vi "Modbus Slave Testbench.vi"() -> ()   [LabVIEW 2021]
uses:
  <vilib>/numeric/Random Number (Range) DBL.vi
  <vilib>/NI/Modbus Library/API/Wrapper/Create TCP Slave.vi
  <vilib>/NI/Modbus Library/API/Slave/Modbus Slave.lvclass
  <vilib>/NI/Modbus Library/API/Wrapper/API Main.lvlib
panel:
  in  "Heatsink Temp (P00022)":u16
  in  "Drive State (P00006)":u16
  in  "DC Link Voltage (P00004)":u16
  in  "Alarm (P00030)":u16
  in  "Fault (P00035)":u16
  out "Fault Reset":u16
  out "Active Mode P00202":enum16{"Nothing", "Torque", "Speed"}(ring)
  out "Command_AO_Reg Setpoint":i16
  out "P00101 Decel":u16
  out "P00100 Accel":u16
  out "Drive Enabled (P00099)":bool
  in  "stop":bool
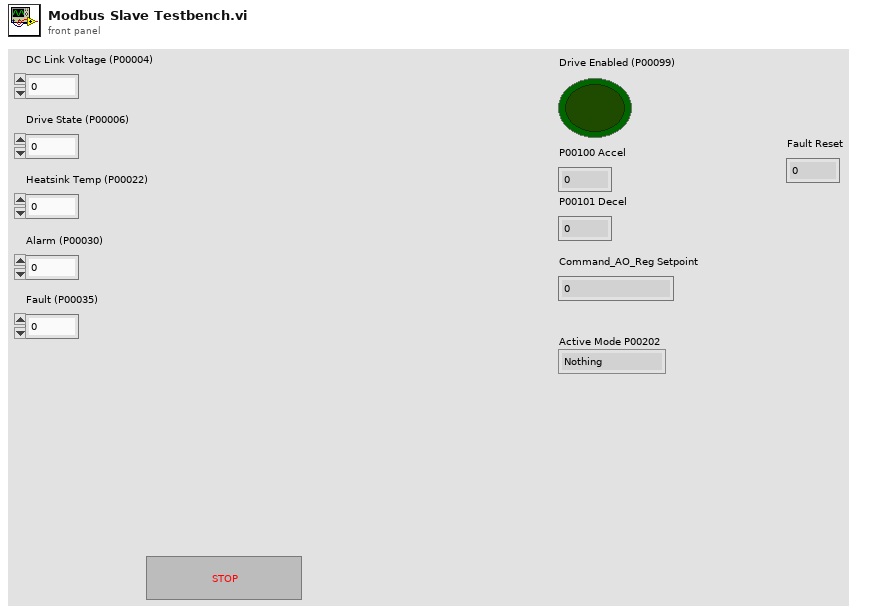
[diagram p1: front panel]
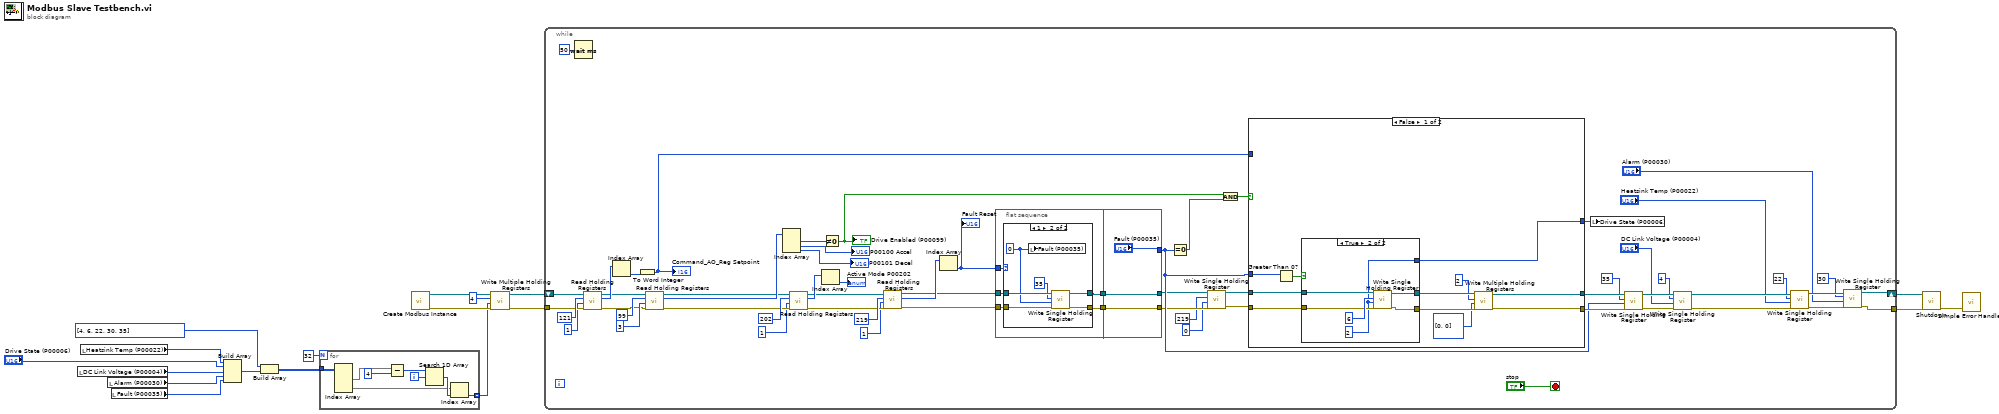
[diagram p0: block diagram]
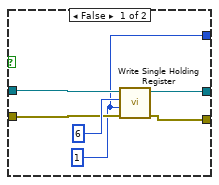
[diagram p3: hidden frame]
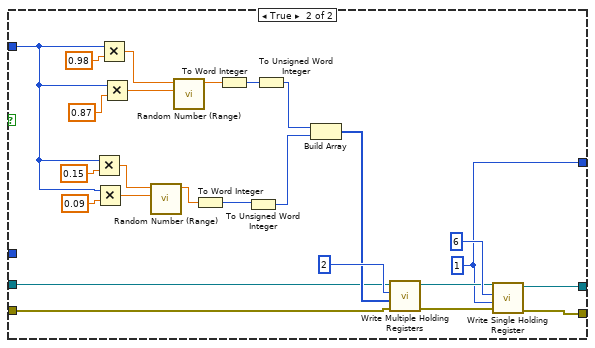
[diagram p4: hidden frame]
diagram:
  n1 = local read "DC Link Voltage (P00004)"() -> (w7:u16)
  n2 = local read "Heatsink Temp (P00022)"() -> (w8:u16)
  n3 = local read "Alarm (P00030)"() -> (w6:u16)
  n4 = local read "Fault (P00035)"() -> (w5:u16)
  n5 = Build Array(w8, "Drive State (P00006)", w7, w6, w5) -> (w3:u16[])
  n6 = Build Array(u16[] [4, 6, 22, 30, 35] ("Simulation Fault"), w3) -> (w2:u16[][])
  n7 = for {
    N: 32 -> [_]
    tunnel: w2 -> [w26]
    tunnel: [w21] -> w12 mode=indexing
    i -> [w24]
    n8 = Index Array(array=w26) -> (element #1=w25:u16[], element #2=w22:u16[])  [unwired: 4 in]
    n9 = Subtract(x=w25, y=4 ("starting address")) -> (x-y=w20:i32[])
    n10 = Search 1D Array(1D array=w20, element=w24) -> (index of element=w23:i32)  [unwired: 1 in]
    n11 = Index Array(array=w22, index=w23) -> (element=w21:u16)
  }
  n12 = call-poly <vilib>:"Create Modbus Instance.vi"() -> ("error out"=w17:errorcluster, "TCP slave instance"=w18:refnum<class "Modbus Slave.lvclass">)  [unwired: 10 in]
  n13 = call-dynamic "Write Multiple Holding Registers.vi"("error in"=w17, "registers to write"=w12, "starting address"=u16 4, "Modbus slave in"=w18) -> ("error out"=w15:errorcluster, "Modbus slave out"=w16:refnum<class "Modbus Slave.lvclass">)  [unwired: 6 in]
  n14 = while {
    tunnel: w15 -> [w65]
    shift-right: [w44] -> w11
    shift-left: w16 -> [w66]
    tunnel: [w45] -> w9
    stop <- "stop" stop-if-true
    n15 = Wait (ms)(milliseconds to wait=u32 50) -> ()  [unwired: 1 out]
    n16 = call-dynamic "Read Holding Registers.vi"("error in"=w65, "number of inputs"=u16 1, "starting address"=u16 121, "Modbus slave in"=w66) -> ("error out"=w64:errorcluster, "register values"=w78:u16[], "Modbus slave out"=w62:refnum<class "Modbus Slave.lvclass">)  [unwired: 5 in]
    n17 = Index Array(array=w78) -> (element=w77:u16)  [unwired: 1 in]
    n18 = To Word Integer(number=w77) -> (16bit integer=w67:i16)
    "Command_AO_Reg Setpoint" <- w67
    n19 = call-dynamic "Read Holding Registers.vi"("error in"=w64, "number of inputs"=u16 3, "starting address"=u16 99, "Modbus slave in"=w62) -> ("error out"=w61:errorcluster, "register values"=w84:u16[], "Modbus slave out"=w63:refnum<class "Modbus Slave.lvclass">)  [unwired: 5 in]
    n20 = Index Array(array=w84) -> (element #1=w83:u16, element #2=→"P00100 Accel":u16, element #3=→"P00101 Decel":u16)  [unwired: 3 in]
    n21 = call-dynamic "Read Holding Registers.vi"("error in"=w61, "number of inputs"=u16 1, "starting address"=u16 202, "Modbus slave in"=w63) -> ("error out"=w59:errorcluster, "register values"=w75:u16[], "Modbus slave out"=w60:refnum<class "Modbus Slave.lvclass">)  [unwired: 5 in]
    n22 = Index Array(array=w75) -> (element=→"Active Mode P00202":u16)  [unwired: 1 in]
    n23 = Not Equal To 0?(x=w83) -> (x != 0?=w70:bool)
    "Drive Enabled (P00099)" <- w70
    n24 = call-dynamic "Read Holding Registers.vi"("error in"=w59, "number of inputs"=u16 1, "starting address"=u16 219, "Modbus slave in"=w60) -> ("error out"=w36:errorcluster, "register values"=w72:u16[], "Modbus slave out"=w37:refnum<class "Modbus Slave.lvclass">)  [unwired: 5 in]
    n25 = Index Array(array=w72) -> (element=w71:u16)  [unwired: 1 in]
    "Fault Reset" <- w71
    n26 = flat-sequence {
      tunnel: w71 -> [w92]
      tunnel: w37 -> [w91]
      tunnel: w36 -> [w90]
      tunnel: [w89] -> w35
      tunnel: [w88] -> w34
      tunnel: ["Fault (P00035)"] -> w38
      tunnel: [w102] -> w29
      tunnel: w35 -> [w102]
      tunnel: [w101] -> w30
      tunnel: w34 -> [w101]
      frame #0 {
        n27 = case shown="1" w92 {
          tunnel: w91 -> [w94 w100]
          tunnel: w90 -> [w93 w99]
          tunnel: [w93 w96] -> w88
          tunnel: [w94 w95] -> w89
          frame 0, Default {
          }
          frame 1 {
            w97 = u16 0 ("Fault (P00035)")
            n28 = local write "Fault (P00035)"(w97) -> ()
            n29 = call-dynamic "Write Single Holding Register.vi"("error in"=w99, "register to write"=w97, "address"=u16 35, "Modbus slave in"=w100) -> ("error out"=w96:errorcluster, "Modbus slave out"=w95:refnum<class "Modbus Slave.lvclass">)  [unwired: 6 in]
          }
        }
      }
      frame #1 {
      }
    }
    n30 = Equal To 0?(x=w38) -> (x = 0?=w69:bool)
    n31 = call-dynamic "Write Single Holding Register.vi"("error in"=w30, "register to write"=u16 0, "address"=u16 219, "Modbus slave in"=w29) -> ("error out"=w31:errorcluster, "Modbus slave out"=w32:refnum<class "Modbus Slave.lvclass">)  [unwired: 6 in]
    n32 = And(x=w70, y=w69) -> (x .and. y?=w68:bool)
    n33 = case shown="False" w68 {
      tunnel: w67 -> [_ w128]
      tunnel: w32 -> [w114 w133]
      tunnel: w31 -> [w113 w132]
      tunnel: [w106 w138] -> w58
      tunnel: [w105 w129] -> w57
      tunnel: w38 -> [w112 _]
      tunnel: [w104 w127] -> w33
      frame False {
        n34 = Greater Than 0?(x=w112) -> (x > 0?=w111:bool)
        n35 = case shown="True" w111 {
          tunnel: w114 -> [w119 w125]
          tunnel: w113 -> [w116 w124]
          tunnel: [w117 w123] -> w109
          tunnel: [w118 w122] -> w110
          tunnel: [w115 w121] -> w104
          frame False {
            w115 = u16 1 ("register to write")
            n36 = call-dynamic "Write Single Holding Register.vi"("error in"=w116, "register to write"=w115, "address"=u16 6, "Modbus slave in"=w119) -> ("error out"=w117:errorcluster, "Modbus slave out"=w118:refnum<class "Modbus Slave.lvclass">)  [unwired: 6 in]
          }
          frame True {
            w121 = u16 2 ("register to write")
            n37 = call-dynamic "Write Single Holding Register.vi"("error in"=w124, "register to write"=w121, "address"=u16 6, "Modbus slave in"=w125) -> ("error out"=w123:errorcluster, "Modbus slave out"=w122:refnum<class "Modbus Slave.lvclass">)  [unwired: 6 in]
          }
        }
        n38 = call-dynamic "Write Multiple Holding Registers.vi"("error in"=w109, "registers to write"=u16[] [0, 0], "starting address"=u16 2 ("address"), "Modbus slave in"=w110) -> ("error out"=w106:errorcluster, "Modbus slave out"=w105:refnum<class "Modbus Slave.lvclass">)  [unwired: 6 in]
      }
      frame True {
        w127 = u16 1 ("register to write")
        n39 = Multiply(x=w128, y=0.15) -> (x*y=w144:dbl)
        n40 = Multiply(x=w128, y=0.09) -> (x*y=w145:dbl)
        n41 = Multiply(x=w128, y=0.98) -> (x*y=w149:dbl)
        n42 = Multiply(x=w128, y=0.87) -> (x*y=w148:dbl)
        n43 = call-poly <vilib>:"Random Number (Range).vi"("lower bound (0)"=w145, "upper bound (100)"=w144) -> ("number"=w140:dbl)  [unwired: 9 in]
        n44 = call-poly <vilib>:"Random Number (Range).vi"("lower bound (0)"=w148, "upper bound (100)"=w149) -> ("number"=w147:dbl)  [unwired: 9 in]
        n45 = To Word Integer(number=w140) -> (16bit integer=w141:i16)
        n46 = To Word Integer(number=w147) -> (16bit integer=w146:i16)
        n47 = To Unsigned Word Integer(number=w141) -> (unsigned 16bit integer=w135:u16)
        n48 = To Unsigned Word Integer(number=w146) -> (unsigned 16bit integer=w136:u16)
        n49 = Build Array(w136, w135) -> (w134:u16[])
        n50 = call-dynamic "Write Multiple Holding Registers.vi"("error in"=w132, "registers to write"=w134, "starting address"=u16 2, "Modbus slave in"=w133) -> ("error out"=w130:errorcluster, "Modbus slave out"=w131:refnum<class "Modbus Slave.lvclass">)  [unwired: 6 in]
        n51 = call-dynamic "Write Single Holding Register.vi"("error in"=w130, "register to write"=w127, "address"=u16 6, "Modbus slave in"=w131) -> ("error out"=w138:errorcluster, "Modbus slave out"=w129:refnum<class "Modbus Slave.lvclass">)  [unwired: 6 in]
      }
    }
    n52 = local write "Drive State (P00006)"(w33) -> ()
    n53 = call-dynamic "Write Single Holding Register.vi"("error in"=w58, "register to write"=w38, "address"=u16 35, "Modbus slave in"=w57) -> ("error out"=w54:errorcluster, "Modbus slave out"=w55:refnum<class "Modbus Slave.lvclass">)  [unwired: 6 in]
    n54 = call-dynamic "Write Single Holding Register.vi"("error in"=w54, "register to write"="DC Link Voltage (P00004)", "address"=u16 4, "Modbus slave in"=w55) -> ("error out"=w50:errorcluster, "Modbus slave out"=w51:refnum<class "Modbus Slave.lvclass">)  [unwired: 6 in]
    n55 = call-dynamic "Write Single Holding Register.vi"("error in"=w50, "register to write"="Heatsink Temp (P00022)", "address"=u16 22, "Modbus slave in"=w51) -> ("error out"=w46:errorcluster, "Modbus slave out"=w47:refnum<class "Modbus Slave.lvclass">)  [unwired: 6 in]
    n56 = call-dynamic "Write Single Holding Register.vi"("error in"=w46, "register to write"="Alarm (P00030)", "address"=u16 30, "Modbus slave in"=w47) -> ("error out"=w45:errorcluster, "Modbus slave out"=w44:refnum<class "Modbus Slave.lvclass">)  [unwired: 6 in]
  }
  n57 = call-dynamic "Shutdown.vi"("error in"=w9, "Modbus slave in"=w11) -> ("error out"=w10:errorcluster)  [unwired: 9 in]
  n58 = call <vilib>:"Simple Error Handler.vi"("error in (no error)"=w10) -> ()  [unwired: 4 in, 5 out]
